vi "VIH ProjFile - Item Rule - Read.vi"(7 "Project Folder":path, 8 "error in":errorcluster, 11 "XML Item":refnum<k20>) -> (0 "error out":errorcluster, 1 "Item Rule out":T1, 2 "Item Path":path, 3 "dup XML Item":refnum<k20>)   [LabVIEW 2014]
doc: "::: VI Helpeks :::\nCopyright (c) 2000-2026 Konstantin Shifershteyn. All rights reserved."
uses:
  _VIH HelpGen.llb/VIH HelpGen Typedef - Cluster - File Rule.ctl
  _VIH HelpGen.llb/VIH HelpGen Typedef - Enum - Default,Enable,Disable.ctl
  _VIH HelpGen.llb/VIH HelpGen Typedef - Cluster - File Rule - Source Paths.ctl
  _VIH HelpGen.llb/VIH HelpGen Typedef - Cluster - File Rule - Target Paths.ctl
  _VIH HelpGen.llb/VIH HelpGen Typedef - Enum - Description Mode.ctl
  _VIH HelpGen.llb/VIH HelpGen Typedef - Cluster - Control Rule.ctl
  _VIH HelpGen.llb/VIH HelpGen Typedef - Cluster - Enum Value Info.ctl
  _VIH HelpGen.llb/VIH HelpGen Typedef - Cluster - Group Rule - Flags.ctl
  <vilib>/xml/Close Reference(Node).vi
  <vilib>/xml/NI_XML.lvlib
  <resource>/objmgr/DOMUserDefRef.rc
panel:
  in  "Item Rule (data)":T1
  # "VI Helpeks\nCopyright (c) 2012-2026 Konstantin Shifershteyn"
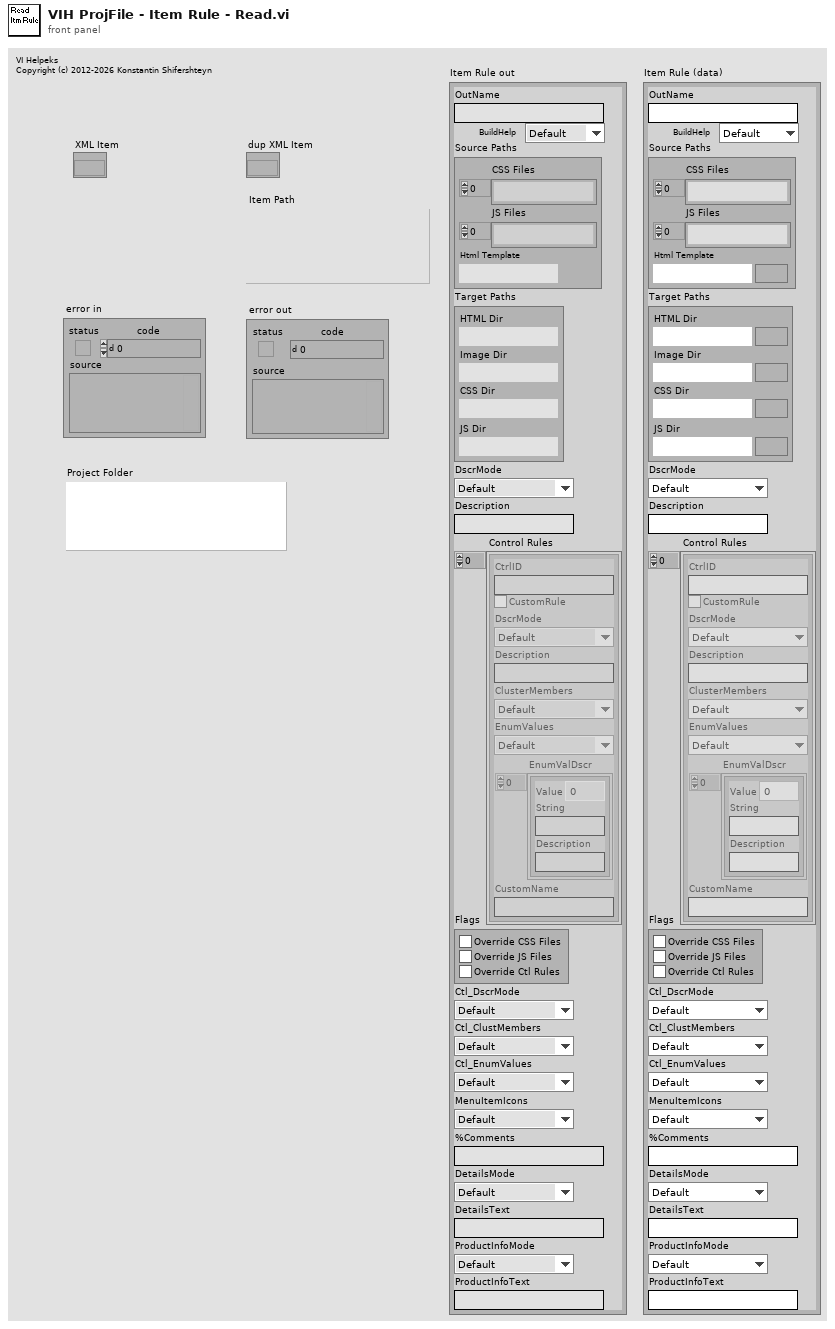
[diagram p1: front panel]
types:
  T1 = typedef "VIH HelpGen Typedef - Cluster - File Rule.ctl" = cluster{"OutName":string, "BuildHelp":T2, "Source Paths":T3, "Target Paths":T4, "DscrMode":T5, "Description":string, "Control Rules":T6[], "Flags":T8, "Ctl_DscrMode":T5, "Ctl_ClustMembers":T2, "Ctl_EnumValues":T2, "MenuItemIcons":T2, "%Comments":string, "DetailsMode":T5, "DetailsText":string, "ProductInfoMode":T2, "ProductInfoText":string}
  T2 = typedef "VIH HelpGen Typedef - Enum - Default,Enable,Disable.ctl" = enum16{"Default", "Enable", "Disable"}
  T3 = typedef "VIH HelpGen Typedef - Cluster - File Rule - Source Paths.ctl" = cluster{"CSS Files":path[], "JS Files":path[], "Html Template":path}
  T4 = typedef "VIH HelpGen Typedef - Cluster - File Rule - Target Paths.ctl" = cluster{"HTML Dir":path, "Image Dir":path, "CSS Dir":path, "JS Dir":path}
  T5 = typedef "VIH HelpGen Typedef - Enum - Description Mode.ctl" = enum16{"Default", "Description", "Description1", "Description2", "Custom", "None"}
  T6 = typedef "VIH HelpGen Typedef - Cluster - Control Rule.ctl" = cluster{"CtrlID":string, "CustomRule":bool, "DscrMode":T5, "Description":string, "ClusterMembers":T2, "EnumValues":T2, "EnumValDscr":T7[], "CustomName":string}
  T7 = typedef "VIH HelpGen Typedef - Cluster - Enum Value Info.ctl" = cluster{"Value":ext, "String":string, "Description":string}
  T8 = typedef "VIH HelpGen Typedef - Cluster - Group Rule - Flags.ctl" = cluster{"Override CSS Files":bool, "Override JS Files":bool, "Override Ctl Rules":bool}
  T9 = typedef "KS HelpGen Typedef - Cluster - File Rule.ctl" = cluster{"OutName":string, "BuildHelp":T10, "Source Paths":T11, "Target Paths":T12, "DscrMode":T13, "Description":string, "Control Rules":T14[], "Flags":T16, "Ctl_DscrMode":T13, "Ctl_ClustMembers":T10, "Ctl_EnumValues":T10, "MenuItemIcons":T10, "%Comments":string, "DetailsMode":T13, "DetailsText":string, "ProductInfoMode":T10, "ProductInfoText":string}
  T10 = typedef "KS HelpGen Typedef - Enum - Default,Enable,Disable.ctl" = enum16{"Default", "Enable", "Disable"}
  T11 = typedef "KS HelpGen Typedef - Cluster - File Rule - Source Paths.ctl" = cluster{"CSS Files":path[], "JS Files":path[], "Html Template":path}
  T12 = typedef "KS HelpGen Typedef - Cluster - File Rule - Target Paths.ctl" = cluster{"HTML Dir":path, "Image Dir":path, "CSS Dir":path, "JS Dir":path}
  T13 = typedef "KS HelpGen Typedef - Enum - Description Mode.ctl" = enum16{"Default", "Description", "Description1", "Description2", "Custom", "None"}
  T14 = typedef "KS HelpGen Typedef - Cluster - Control Rule.ctl" = cluster{"CtrlID":string, "CustomRule":bool, "DscrMode":T13, "Description":string, "ClusterMembers":T10, "EnumValues":T10, "EnumValDscr":T15[], "CustomName":string}
  T15 = typedef "KS HelpGen Typedef - Cluster - Enum Value Info.ctl" = cluster{"Value":ext, "String":string, "Description":string}
  T16 = typedef "KS HelpGen Typedef - Cluster - Group Rule - Flags.ctl" = cluster{"Override CSS Files":bool, "Override JS Files":bool, "Override Ctl Rules":bool}
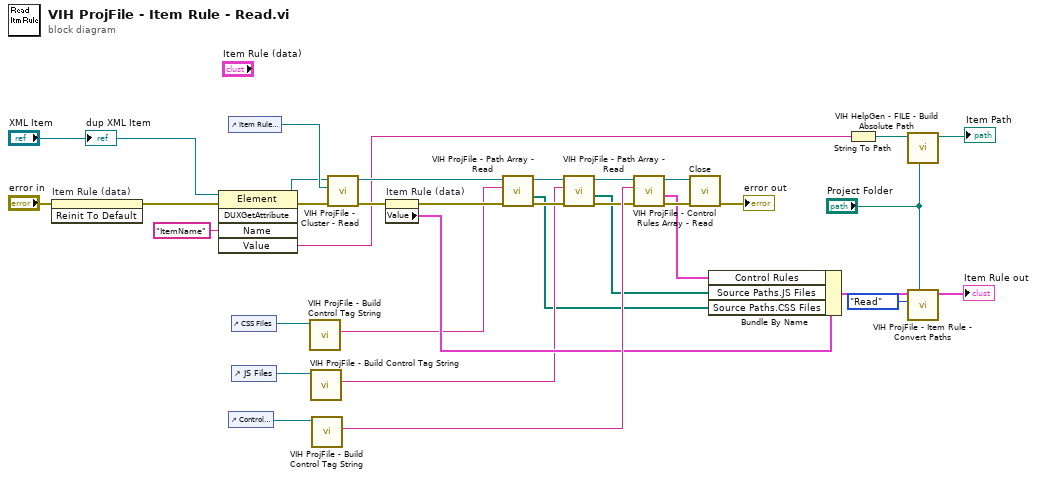
[diagram p0: block diagram]
diagram:
  n1 = invoke on="Item Rule (data)" class="Clust (strict)" method="Reinit To Default"(error in="error in") -> (error out=w11:errorcluster)  [unwired: 2 in, 2 out]
  n2 = invoke class="Element" method="DUXGetAttribute"(reference="XML Item", error in=w11, "Name"="ItemName") -> (reference out=w8:refnum<k20>, error out=w10:errorcluster, "Value"=w2:string)  [unwired: 2 in, 2 out]
  n3 = control-ref of="Item Rule (data)"() -> (w34:refnum<vi>)
  n4 = control-ref of="Control Rules"() -> (w13:refnum<vi>)
  n5 = control-ref of="CSS Files"() -> (w15:refnum<vi>)
  n6 = control-ref of="JS Files"() -> (w14:refnum<vi>)
  n7 = call "VIH ProjFile - Build Control Tag String.vi"("Ctl Refnum"=w15) -> ("Control Tag"=w19:string)  [unwired: 6 in, 4 out]
  n8 = call "VIH ProjFile - Build Control Tag String.vi"("Ctl Refnum"=w14) -> ("Control Tag"=w18:string)  [unwired: 6 in, 4 out]
  n9 = call "VIH ProjFile - Build Control Tag String.vi"("Ctl Refnum"=w13) -> ("Control Tag"=w30:string)  [unwired: 6 in, 4 out]
  n10 = call "VIH ProjFile - Cluster - Read.vi"("error in"=w10, "Ctl Refnum"=w34, "XML Parent Item"=w8) -> ("error out"=w28:errorcluster, "dup XML Parent Item"=w25:refnum<k20>)  [unwired: 7 in]
  n11 = property on="Item Rule (data)" class="Clust (strict)"(error in=w28) -> (error out=w22:errorcluster, "Value"=w27:T9)  [unwired: 1 in, 1 out]
  n12 = call "VIH ProjFile - Path Array - Read.vi"("error in"=w22, "Property Name"=w19, "XML Parent Item"=w25) -> ("error out"=w21:errorcluster, "Files"=w16:path[], "dup XML Parent Item"=w24:refnum<k20>)  [unwired: 6 in]
  n13 = call "VIH ProjFile - Path Array - Read.vi"("error in"=w21, "Property Name"=w18, "XML Parent Item"=w24) -> ("error out"=w20:errorcluster, "Files"=w17:path[], "dup XML Parent Item"=w23:refnum<k20>)  [unwired: 6 in]
  n14 = call "VIH ProjFile - Control Rules Array - Read.vi"("error in"=w20, "Property Name"=w30, "XML Parent Item"=w23) -> ("error out"=w31:errorcluster, "Control Rules"=w26:T6[], "dup XML Parent Item"=w32:refnum<k20>)  [unwired: 5 in, 1 out]
  n15 = call-poly <vilib>:"Close.vi"("error in (no error)"=w31, "node"=w32) -> ("error out"=→"error out":errorcluster)  [unwired: 7 in]
  n16 = Bundle By Name(cluster=w27, "Control Rules"=w26, "Source Paths.JS Files"=w17, "Source Paths.CSS Files"=w16) -> (w7:T9)
  n17 = String To Path(string=w2) -> (path=w3:path)
  n18 = call "VIH HelpGen - FILE - Build Absolute Path.vi"("Root Path"="Project Folder", "Path in"=w3) -> ("Path out"=→"Item Path":path)  [unwired: 9 in]
  n19 = call "VIH ProjFile - Item Rule - Convert Paths.vi"("Root Dir"="Project Folder", "Operation"=enum16{"Read", "Write"}."Read", "Item Rule"=w7) -> ("Item Rule out"=→"Item Rule out":T1)  [unwired: 8 in]
  "dup XML Item" <- "XML Item"
